vi "test_prompt_with_arguments.vi"(8 "error in":errorcluster, 10 "arg2":string, 11 "arg1":string) -> (0 "error out":errorcluster, 3 "prompt":string)   [LabVIEW 2020, in "Conformance MCP Server.lvlib"]
doc: "Conformance fixture (scenario prompts-get-with-args). A prompt with the two required arguments arg1 and arg2 that returns the text \"Prompt with arguments: arg1='<arg1>', arg2='<arg2>'\"."
uses:
  Conformance MCP Server.lvlib
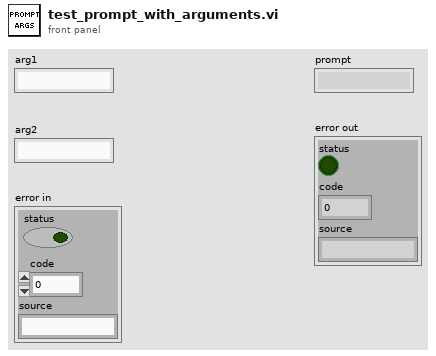
[diagram p1: front panel]
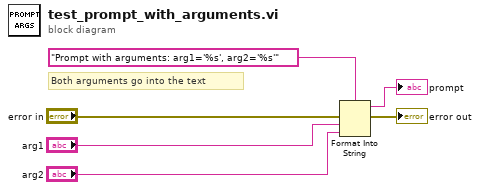
[diagram p0: block diagram]
diagram:
  # "Both arguments go into the text"
  n1 = Format Into String(format string="Prompt with arguments: arg1='%s', arg2='%s'", error in="error in", "arg1", "arg2") -> (resulting string=→"prompt":string, error out=→"error out":errorcluster)  [unwired: 1 in]
